vi "Set Resistance Colors.vi"(4 "Selec":T2) -> (1 "Color":T1)   [LabVIEW 2018, in "Resistance Colors.lvlib"]
doc: "Sets the resistor band colors according to the selected resistor parameters.\n\nThe VI receives the <b>Selec</b> cluster, containing the selected values for the resistor band digits, multiplier, tolerance, and temperature coefficient.\n\nIt calls the corresponding color converter VIs to obtain the color associated with each parameter and groups the resulting colors into the <b>Color</b> cluster.\n\nThe resulting cluster contains the colors for the first, second, and third significant digits, multiplier, tolerance, and temperature coefficient.\n\nThe VI returns the resulting colors through <b>Color</b>."
uses:
  Resistance Colors.lvlib
  Resistor Controls/Selectors--cluster.ctl
  Resistor Controls/Digit--enum.ctl
  Resistor Controls/Multiplier--enum.ctl
  Resistor Controls/Tolerance--enum.ctl
  Resistor Controls/Temp Coefficient--enum.ctl
  Colors--cluster.ctl
  Resistor Controls/Resistance Controls.lvlib
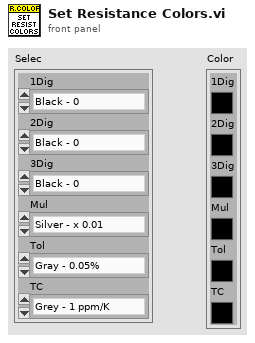
[diagram p1: front panel]
types:
  T1 = typedef "Resistance Colors.lvlib/Colors--cluster.ctl" = cluster{"1Dig":u32, "2Dig":u32, "3Dig":u32, "Mul":u32, "Tol":u32, "TC":u32}
  T2 = typedef "Resistance Controls.lvlib/Selectors--cluster.ctl" = cluster{"1Dig":T3, "2Dig":T3, "3Dig":T3, "Mul":T4, "Tol":T5, "TC":T6}
  T3 = typedef "Resistance Controls.lvlib/Digit--enum.ctl" = enum16{"Black - 0", "Brown - 1", "Red - 2", "Orange - 3", "Yellow - 4", "Green - 5", "Blue - 6", "Violet - 7", "Grey - 8", "White - 9"}
  T4 = typedef "Resistance Controls.lvlib/Multiplier--enum.ctl" = enum16{"Silver - x 0.01", "Gold - x 0.1 ", "Black - x 1", "Brown - x 10", "Red - x 100", "Orange - x 1k", "Yellow - x 10k", "Green - 100k", "Blue - x 1M", "Violet - x10 M", "Grey - x 100M", "White - x 1G"}
  T5 = typedef "Resistance Controls.lvlib/Tolerance--enum.ctl" = enum16{"Gray - 0.05%", "Violet - 0.1%", "Blue - 0.25%", "Green - 0.5%", "Brown - 1%", "Red - 2%", "Gold - 5%", "Silver - 10%", "None - 20%"}
  T6 = typedef "Resistance Controls.lvlib/Temp Coefficient--enum.ctl" = enum16{"Grey - 1 ppm/K", "Violet - 5 ppm/K", "Blue - 10 ppm/K", "Green - 20 ppm/K", "Yellow - 25 ppm/K", "Orange - 15 ppm/K", "Red - 50 ppm/K", "Brown - 100 ppm/K", "Black - 250 ppm/K"}
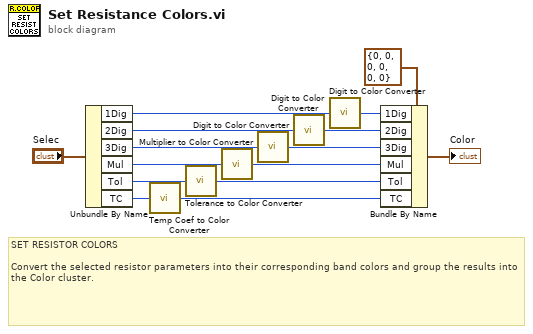
[diagram p0: block diagram]
diagram:
  # "SET RESISTOR COLORS\n\nConvert the selected resistor parameters into their corresponding band colors and group the results into the Color cluster."
  n1 = Unbundle By Name("Selec") -> ("1Dig"=w10:T3, "2Dig"=w11:T3, "3Dig"=w14:T3, "Mul"=w12:T4, "Tol"=w13:T5, "TC"=w15:T6)
  n2 = call "Temp Coef to Color Converter.vi"("Temp Coef select"=w15) -> ("Temp Coef Color"=w3:u32)  [unwired: 6 in]
  n3 = call "Tolerance to Color Converter.vi"("Tolerance select"=w13) -> ("Tolerance Color"=w4:u32)  [unwired: 6 in]
  n4 = call "Multiplier to Color Converter.vi"("Multiplier select"=w12) -> ("Multiplier Color"=w5:u32)  [unwired: 6 in]
  n5 = call "Digit to Color Converter.vi"("Digit select"=w14) -> ("Digit Color"=w6:u32)  [unwired: 4 in]
  n6 = call "Digit to Color Converter.vi"("Digit select"=w11) -> ("Digit Color"=w7:u32)  [unwired: 4 in]
  n7 = call "Digit to Color Converter.vi"("Digit select"=w10) -> ("Digit Color"=w8:u32)  [unwired: 4 in]
  n8 = Bundle By Name(cluster=T1 {"1Dig"=0, "2Dig"=0, "3Dig"=0, "Mul"=0, "Tol"=0, "TC"=0} ("Color"), "1Dig"=w8, "2Dig"=w7, "3Dig"=w6, "Mul"=w5, "Tol"=w4, "TC"=w3) -> (→"Color":T1)
